vi "RemoteVI Capture Frame.vi"(0 "cache":T1, 5 "hWnd":u64) -> (4 "frame":u32[][](array[numeric]), 6 "cache out":T1)   [LabVIEW 2020, in "RemoteVI.lvlib"]
doc: "Makes the image for one frame: the WHOLE front panel window below its title bar - menu bar, toolbar, panel and scrollbars, as the window shows them - which is the window's client area (LabVIEW draws its own menu bar, toolbar and scrollbars inside it). The client area is copied from the window's composited surface (RemoteVI Copy Window.vi: GetDC + BitBlt), which also works while the window is covered or behind an open menu, and does not make LabVIEW draw the window again: 2-5 ms instead of 40-50 ms for the demo with PrintWindow, which also kept LabVIEW's UI thread busy repainting the whole window for every frame (measured). No VI Server call, so it also runs while a popup is open. When the window cannot be copied (minimized, gone) the cache is kept, so the last frame stays."
uses:
  RemoteVI.lvlib
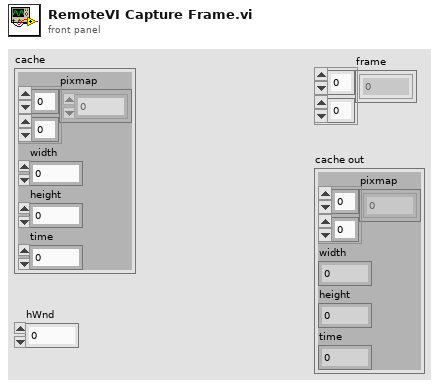
[diagram p1: front panel]
types:
  T1 = cluster{"pixmap":u32[][], "width":i32, "height":i32, "time":u32}
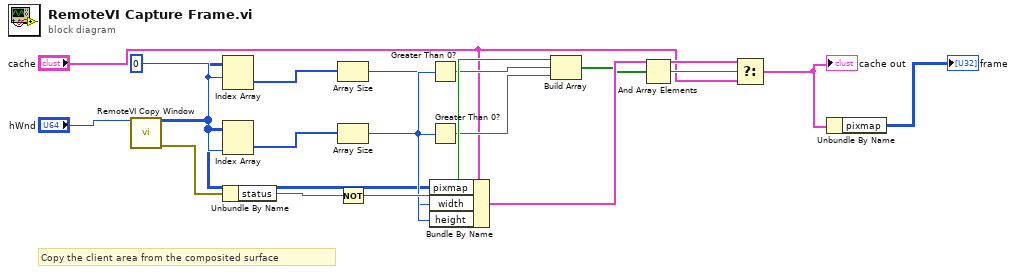
[diagram p0: block diagram]
diagram:
  w5 = 0
  # "Copy the client area from the composited surface"
  n1 = call "RemoteVI Copy Window.vi"("hwnd"="hWnd") -> ("pixmap"=w3:u32[][], "error out"=w4:errorcluster)  [unwired: 13 in]
  n2 = Index Array(array=w3, index (row)=w5) -> (element=w6:u32[])  [unwired: 1 in]
  n3 = Index Array(array=w3, index (col)=w5) -> (element=w7:u32[])  [unwired: 1 in]
  n4 = Unbundle By Name(w4) -> ("status"=w10:bool)
  n5 = Array Size(array=w6) -> (size(s)=w8:i32)
  n6 = Array Size(array=w7) -> (size(s)=w9:i32)
  n7 = Not(x=w10) -> (.not. x?=w13:bool)
  n8 = Greater Than 0?(x=w9) -> (x > 0?=w11:bool)
  n9 = Greater Than 0?(x=w8) -> (x > 0?=w12:bool)
  n10 = Bundle By Name(cluster="cache", "pixmap"=w3, "width"=w8, "height"=w9) -> (w16:T1)
  n11 = Build Array(w13, w11, w12) -> (w14:bool[])
  n12 = And Array Elements(Boolean array=w14) -> (logical AND=w15:bool)
  n13 = Select(t=w16, s=w15, f="cache") -> (s? t:f=w17:T1)
  "cache out" <- w17
  n14 = Unbundle By Name(w17) -> ("pixmap"=→"frame":u32[][])
